vi "Find Scalar Group.vi"(8 "error in":errorcluster, 10 "Group Name":string, 11 "FPGA Addon refnum in":T1 format="%.0x") -> (0 "error out":errorcluster, 1 "Found ?":bool, 2 "Group Scalar Data":T2 {"Scalar Section ref" format="%.0x"; "Group Section ref" format="%.0x"; "Group Scalar Registers"."Data Type" format="%.0x"}, 3 "FPGA Addon refnum out":T1=18446744073709551615 format="%.0x")   [LabVIEW 2020, in "Scripting API.lvlib"]
uses:
  Scripting API.lvlib
  <vilib>/NI VeriStand/Custom Device API/Custom Device Item Ref.ctl
  TypeDefs/Group Scalar Data.ctl
  Addon/Addon Shared/Types/Register Information.ctl
  Addon/Addon Shared/Types/FPGA Addon Data Type.ctl
  Addon/Addon Shared/Types/FG Action.ctl
  Addon/Addon Shared/SubVIs/Constants.vi
  <vilib>/NI/NI VeriStand Advanced SysDef API/_SubVIs/SysDef.Search.GUID.vi
  <vilib>/NI/NI VeriStand Advanced SysDef API/SysDef API/SysDef.Property.Get.vi
  <vilib>/NI/NI VeriStand Advanced SysDef API/_SubVIs/SysDef.Property.Get.Variant.vi
  <vilib>/NI/NI VeriStand Advanced SysDef API/SysDef API/SysDef.Property.Set.vi
  <vilib>/NI/NI VeriStand Advanced SysDef API/_SubVIs/SysDef.Property.Set.Variant.vi
  <vilib>/NI/NI VeriStand Advanced SysDef API/_SubVIs/SysDef.Search.Name.vi
  <vilib>/NI/NI VeriStand Advanced SysDef API/SysDef API/Advanced System Definition.lvlib
  Addon/Addon Shared/FPGA Addon Shared.lvlib
  <vilib>/NI VeriStand/Custom Device API/Custom Device API.lvlib
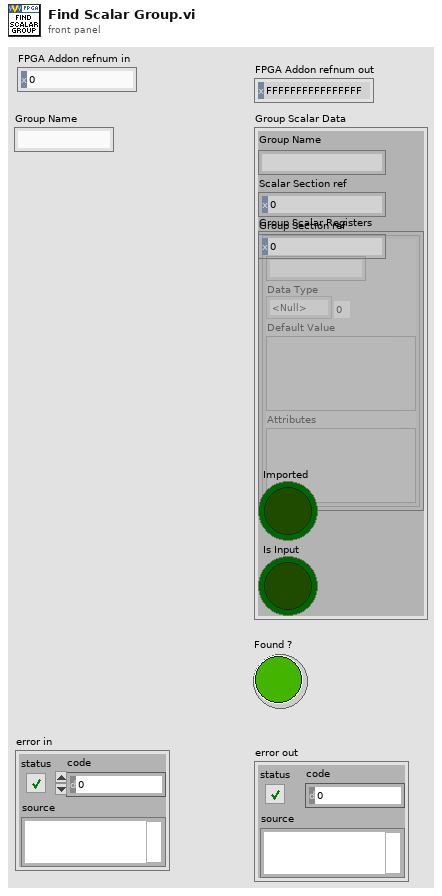
[diagram p1: front panel]
types:
  T1 = typedef "Custom Device API.lvlib/Custom Device Item Ref.ctl" = u64
  T2 = typedef "Scripting API.lvlib/Group Scalar Data.ctl" = cluster{"Group Name":string, "Scalar Section ref":T1, "Group Section ref":T1, "Group Scalar Registers":T3[], "Imported":bool, "Is Input":bool}
  T3 = typedef "FPGA Addon Shared.lvlib/Register Information.ctl" = cluster{"Name":string, "Data Type":T4, "Default Value":variant, "Attributes":variant}
  T4 = typedef "FPGA Addon Shared.lvlib/FPGA Addon Data Type.ctl" = enum8{"<Null>", "I8", "I16", "I32", "I64", "U8", "U16", "U32", "U64", "SGL", "Boolean", "Analog PWM In Settings", "Analog PWM In", "Digital PWM In Settings", "Digital PWM In", "Digital PWM Out", "Sine Out", "FXP", "FXP+/-24.5", "FXP+/-16.5", "FXP+/-32.8", "FXP+/-64.32", "FXP+/-16.7", "FXP+/-20.5", "FXP+/-27.5", "FXP+/-32.16", "FXP+16.3", "FXP+18.3", "Digital Static In", "Digital Static Out", "Digital Static In Settings", "Digital WSS Out", "Quad Encoder Settings", "Quad Encoder In", "Group"}
  T5 = typedef "FPGA Addon Shared.lvlib/FG Action.ctl" = enum8{"GET", "SET"}
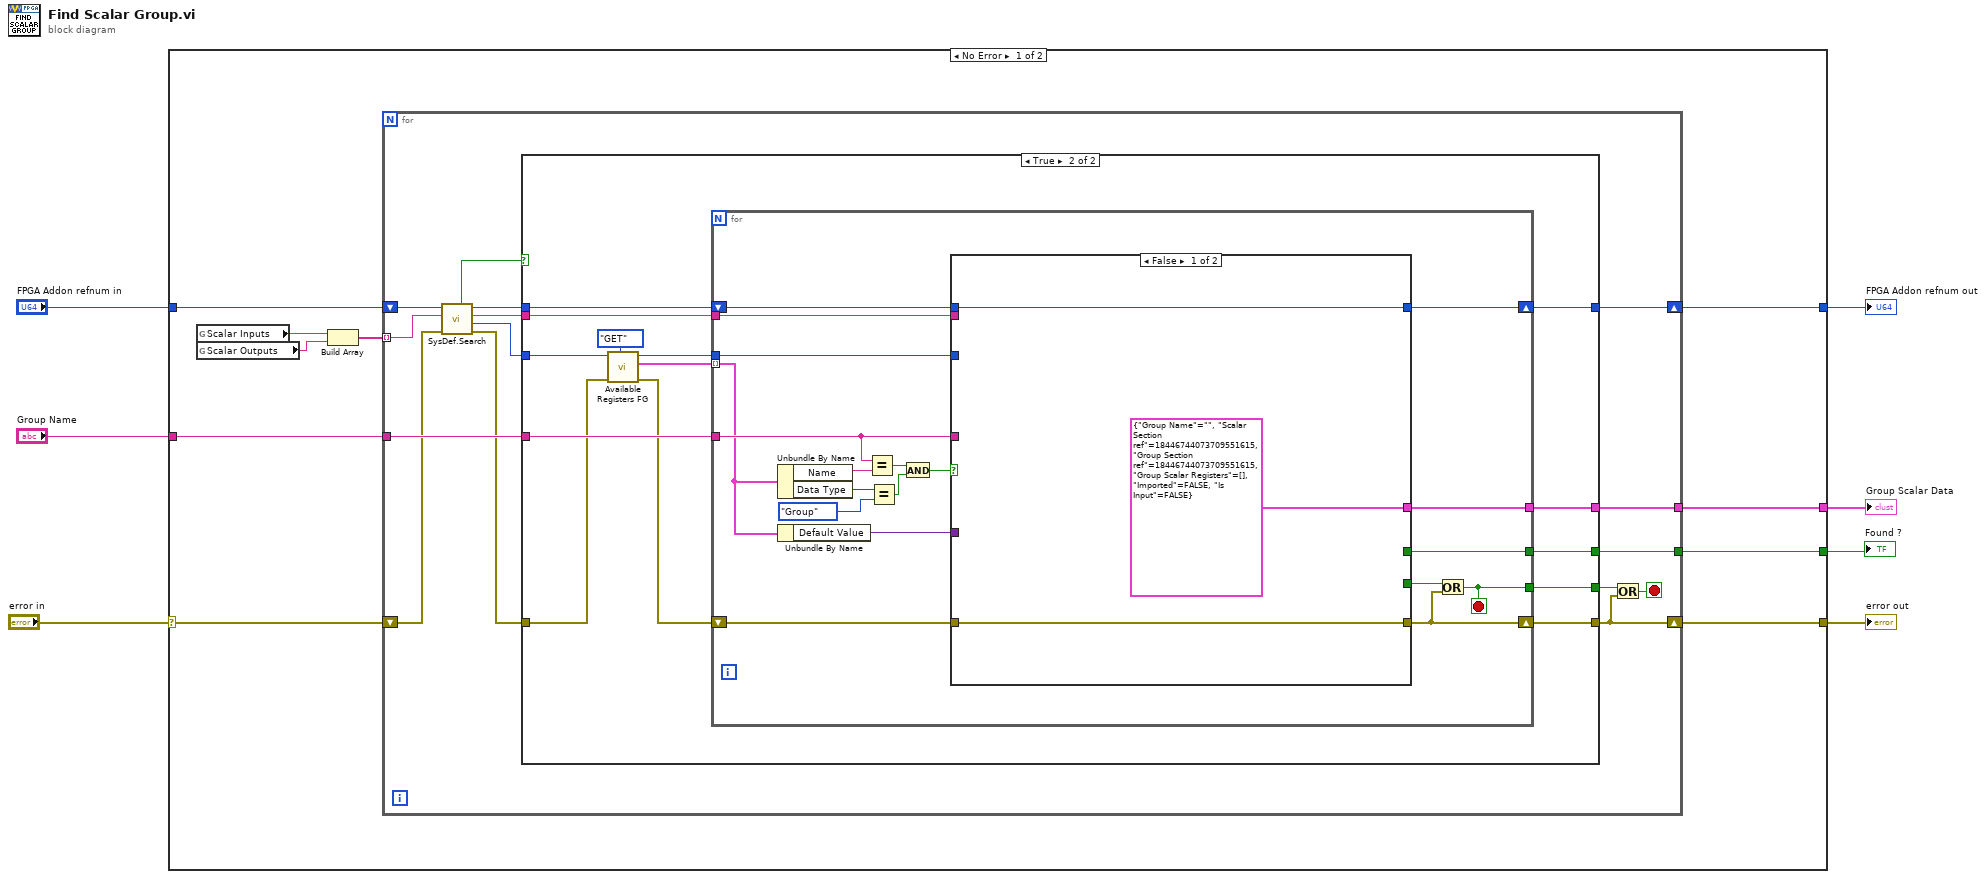
[diagram p0: block diagram]
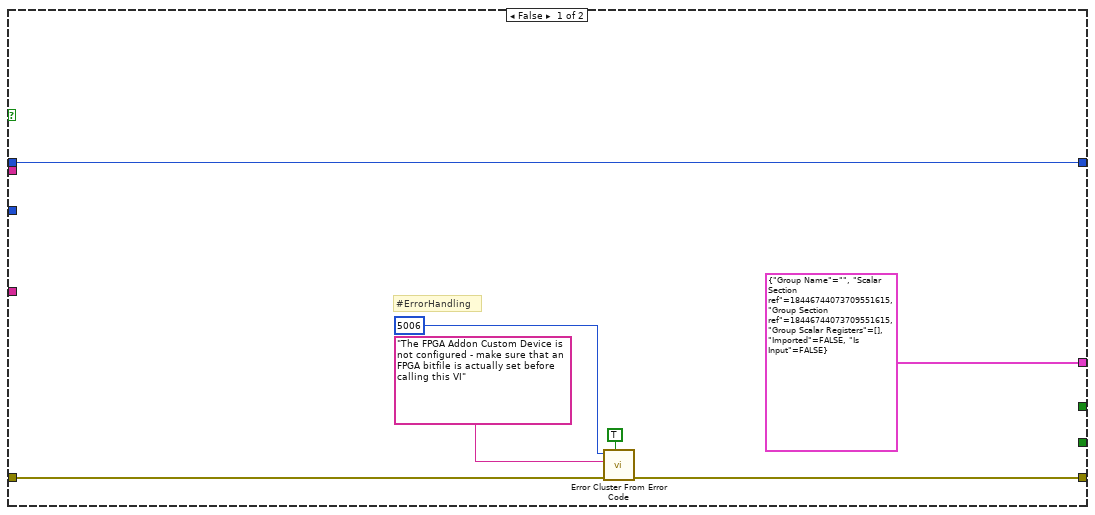
[diagram p2: hidden frame]
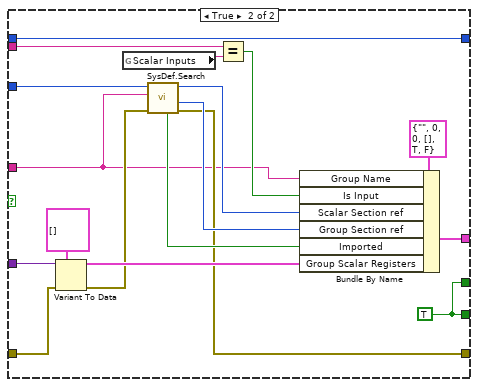
[diagram p3: hidden frame]
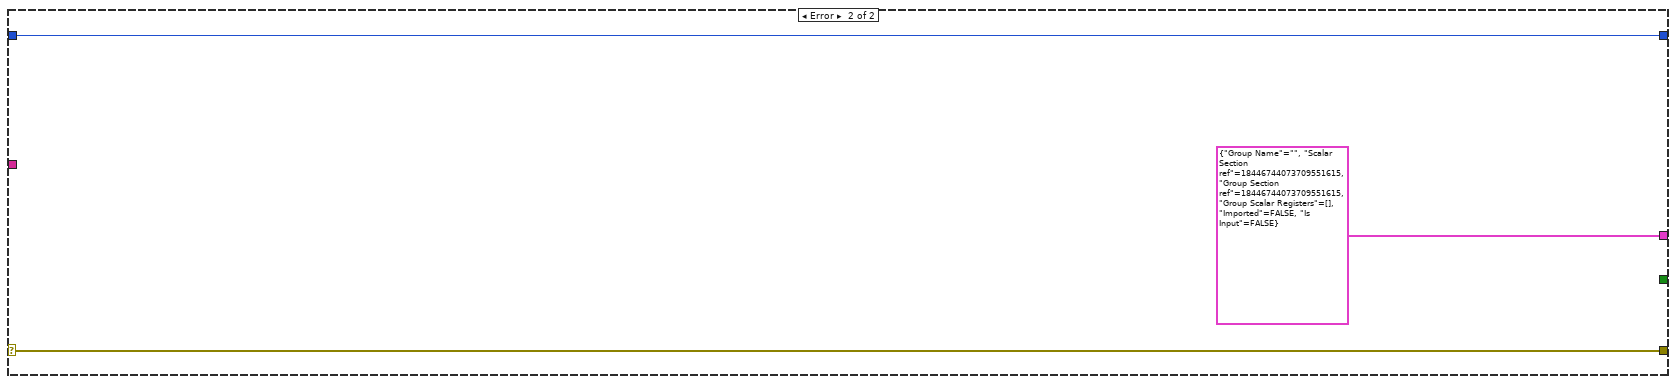
[diagram p4: hidden frame]
diagram:
  n1 = case shown="No Error" "error in" {
    selector: "error in" -> [w12 w95]
    tunnel: "Group Name" -> [w17 _]
    tunnel: "FPGA Addon refnum in" -> [w13 w93]
    tunnel: [w11 w95] -> w4
    tunnel: [w10 T2 {"Group Name"="", "Scalar Section ref"=18446744073709551615, "Group Section ref"=18446744073709551615, "Group Scalar Registers"=[], "Imported"=FALSE, "Is Input"=FALSE}] -> w3
    tunnel: [w9 w93] -> w2
    tunnel: [w8 _] -> w1
    frame No Error {
      n2 = global read "Constants.vi" "Scalar Inputs"() -> (w15:string)
      n3 = global read "Constants.vi" "Scalar Outputs"() -> (w14:string)
      n4 = Build Array(w15, w14) -> (w16:string[])
      n5 = for {
        tunnel: w16 -> [w18] mode=indexing
        tunnel: w17 -> [w29]
        shift-right: [w26] -> w9
        shift-left: w13 -> [w31]
        tunnel: [w25] -> w10
        shift-right: [w22] -> w11
        shift-left: w12 -> [w24]
        tunnel: [w19] -> w8
        stop <- w20 stop-if-true
        n6 = call-poly <vilib>:"SysDef.Search.vi"("error in (no error)"=w24, "GUID"=w18, "nodeID"=w31) -> ("error out"=w23:errorcluster, "Value out"=w30:u64, "nodeID out"=w27:u64, "Found?"=w28:bool)  [unwired: 5 in]
        n7 = case shown="True" w28 {
          tunnel: w30 -> [_ w51]
          tunnel: w29 -> [_ w50]
          tunnel: w27 -> [w38 w47]
          tunnel: [w38 w46] -> w26
          tunnel: [T2 {"Group Name"="", "Scalar Section ref"=18446744073709551615, "Group Section ref"=18446744073709551615, "Group Scalar Registers"=[], "Imported"=FALSE, "Is Input"=FALSE} w45] -> w25
          tunnel: w23 -> [w33 w44]
          tunnel: [_ w42] -> w21
          tunnel: [w32 w41] -> w22
          tunnel: [_ w40] -> w19
          tunnel: w18 -> [_ w39]
          frame False {
            # "#ErrorHandling"
            n8 = call <vilib>:"Error Cluster From Error Code.vi"("show call chain? (False)"=TRUE, "error in (no error)"=w33, "error message (\"\")"="The FPGA Addon Custom Device is not configured - make sure that an FPGA bitfile is actually set before calling this VI" ("error message (\"\")"), "error code (0)"=5006) -> ("error out"=w32:errorcluster)  [unwired: 5 in]
          }
          frame True {
            n9 = call "Available Registers FG.vi"("Action"=FG_Action."GET", "error in (no error)"=w44, "Item Ref"=w51) -> ("error out"=w43:errorcluster, "Available Registers"=w48:T3[], "Item Ref out"=w49:T1)  [unwired: 6 in]
            n10 = for {
              tunnel: w48 -> [w62] mode=indexing
              tunnel: w50 -> [w63]
              tunnel: w49 -> [w68]
              shift-right: [w60] -> w46
              shift-left: w47 -> [w67]
              tunnel: [w59] -> w45
              shift-right: [w55] -> w41
              shift-left: w43 -> [w58]
              tunnel: [w57] -> w42
              tunnel: [w54] -> w40
              tunnel: w39 -> [w53]
              stop <- w57 stop-if-true
              n11 = Unbundle By Name(w62) -> ("Name"=w64:string, "Data Type"=w66:T4)
              n12 = Unbundle By Name(w62) -> ("Default Value"=w61:variant)
              n13 = Equal?(x=w63, y=w64) -> (x = y?=w71:bool)
              n14 = Equal?(x=w66, y=FPGA_Addon_Data_Type."Group" ("x")) -> (x = y?=w70:bool)
              n15 = And(x=w71, y=w70) -> (x .and. y?=w69:bool)
              n16 = case shown="False" w69 {
                tunnel: w68 -> [_ w92]
                tunnel: w67 -> [w74 w85]
                tunnel: w63 -> [_ w75]
                tunnel: w61 -> [_ w88]
                tunnel: [w74 w85] -> w60
                tunnel: [T2 {"Group Name"="", "Scalar Section ref"=18446744073709551615, "Group Section ref"=18446744073709551615, "Group Scalar Registers"=[], "Imported"=FALSE, "Is Input"=FALSE} w84] -> w59
                tunnel: w58 -> [w72 w82]
                tunnel: [w72 w83] -> w55
                tunnel: [_ w79] -> w56
                tunnel: [_ w79] -> w54
                tunnel: w53 -> [_ w78]
                frame False {
                }
                frame True {
                  w79 = TRUE
                  n17 = Variant To Data(error in=w82, type=T3[] [], Variant=w88) -> (data=w86:T3[], error out=w81:errorcluster)
                  n18 = global read "Constants.vi" "Scalar Inputs"() -> (w77:string)
                  n19 = call-poly <vilib>:"SysDef.Search.vi"("error in (no error)"=w81, "Name"=w75, "nodeID"=w92) -> ("error out"=w83:errorcluster, "Value out"=w90:u64, "nodeID out"=w89:u64, "Found?"=w91:bool)  [unwired: 5 in]
                  n20 = Equal?(x=w78, y=w77) -> (x = y?=w76:bool)
                  n21 = Bundle By Name(cluster=T2 {"Group Name"="", "Scalar Section ref"=0, "Group Section ref"=0, "Group Scalar Registers"=[], "Imported"=TRUE, "Is Input"=FALSE}, "Group Name"=w75, "Is Input"=w76, "Scalar Section ref"=w89, "Group Section ref"=w90, "Imported"=w91, "Group Scalar Registers"=w86) -> (w84:T2)
                }
              }
              n22 = Or(x=w56, y=w55) -> (x .or. y?=w57:bool)
            }
          }
        }
        n23 = Or(x=w21, y=w22) -> (x .or. y?=w20:bool)
      }
    }
    frame Error {
    }
  }
  "error out" <- w4
  "Group Scalar Data" <- w3
  "FPGA Addon refnum out" <- w2
  "Found ?" <- w1
